vi "Stop Core.vi"(10 "final error code":i32, 11 "DAQ Timed SPIM in":refnum<class "DAQ Timed SPIM.lvclass">) -> (3 "DAQ Timed SPIM out":refnum<class "DAQ Timed SPIM.lvclass">)   [LabVIEW 2020, in "DAQ Timed SPIM.lvlib" / "DAQ Timed SPIM.lvclass"]
doc: "(<B>Filename</B>: Actor Framework.lvlib:Actor.lvclass:Stop Core.vi)\n\nDefines what the actor does before it stops. Use the <B>final error code</B> input to determine whether the actor shut down in response to an error.\n\nBy default, this method passes the Stop message along to all auto-stop nested actors. A descendant class may override this method to define additional behavior, such as shutting down any processes the actor initiated in its override of the Actor Core method."
uses:
  DAQ Timed SPIM.lvclass
  <vilib>/ActorFramework/Actor/Actor.lvclass
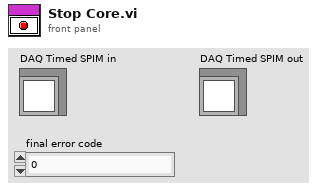
[diagram p1: front panel]
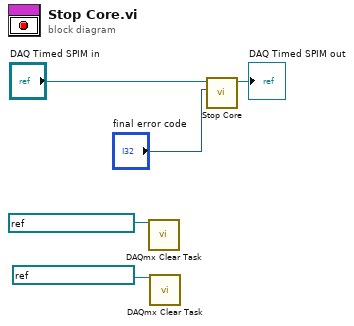
[diagram p0: block diagram]
diagram:
  n1 = call <vilib>:"DAQmx Clear Task.vi"("task in"=refnum<k21> "SPIM_Analog_Task") -> ()  [unwired: 14 in, 1 out]
  n2 = call <vilib>:"DAQmx Clear Task.vi"("task in"=refnum<k21> "SPIM_Digital_Task") -> ()  [unwired: 14 in, 1 out]
  n3 = call-parent "Stop Core.vi"("final error code"="final error code", "Actor in"="DAQ Timed SPIM in") -> ("Actor out"=→"DAQ Timed SPIM out":refnum<class "DAQ Timed SPIM.lvclass">)  [unwired: 9 in]
